vi "child.vi"   [LabVIEW 2020]
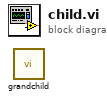
[diagram p0: block diagram]
diagram:
  n1 = call "grandchild.vi"() -> ()  [unwired: 1 in]
